vi "setUp.vi"(8 "error in (no error)":errorcluster, 11 "reference in":refnum<class "Instrument Addon Error System Tests.lvclass">) -> (0 "error out":errorcluster, 3 "reference out":refnum<class "Instrument Addon Error System Tests.lvclass">)   [LabVIEW 2020, in "Instrument Addon Error System Tests.lvclass"]
doc: "setUp runs prior to the test method during test execution. Use this method to initialize any object data required by your tests."
uses:
  Instrument Addon Error System Tests.lvclass
  C:/Program Files (x86)/National Instruments/LabVIEW 2020/vi.lib/NI/VeriStand Custom Device Testing Tools/VeriStandTestCase/VeriStandTestCase.lvclass
  C:/Program Files (x86)/National Instruments/LabVIEW 2020/vi.lib/addons/_JKI Toolkits/VI Tester/TestCase.llb/TestCase.lvclass
  <vilib>/addons/_JKI Toolkits/VI Tester/TestCase.llb/TestCase.lvclass
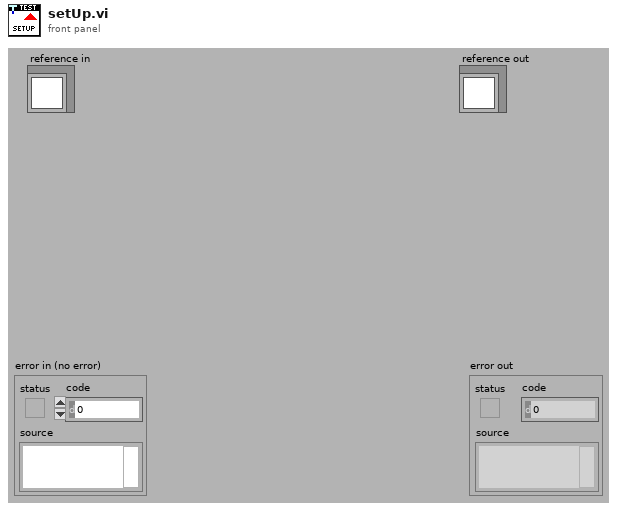
[diagram p1: front panel]
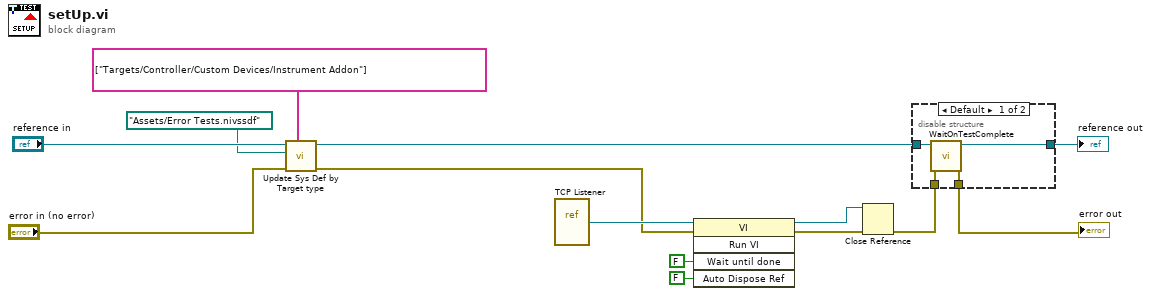
[diagram p0: block diagram]
diagram:
  n1 = call "Update Sys Def by Target type.vi"("nodepaths"=string[] ["Targets/Controller/Custom Devices/Instrument Addon"], "error in (no error)"="error in (no error)", "Sys Def relative path:"=path "Assets/Error Tests.nivssdf", "VeriStandTestCase in"="reference in") -> ("error out"=w3:errorcluster, "VeriStandTestCase out"=w5:refnum<class "Instrument Addon Error System Tests.lvclass">)  [unwired: 6 in]
  n2 = vi-ref "TCP Listener.vi"() -> (w12:refnum<vi>)
  n3 = invoke class="VI" method="Run VI"(reference=w12, error in=w3, "Wait until done"=FALSE ("Wait Until Done"), "Auto Dispose Ref"=FALSE ("Auto Dispose Reference")) -> (reference out=w11:refnum<vi>, error out=w10:errorcluster)  [unwired: 1 in, 3 out]
  n4 = Close Reference(reference=w11, error in (no error)=w10) -> (error out=w9:errorcluster)
  n5 = disable-structure shown="Default" {
    disable-tunnel: w9 -> [w18 w19]
    disable-tunnel: [w17 w19] -> w14
    disable-tunnel: [w16 w20] -> w13
    disable-tunnel: w5 -> [w15 w20]
    frame condition #0 (active) {
      n6 = call <vilib>:"WaitOnTestComplete.vi"("error in (no error)"=w18, "TestCase in"=w15) -> ("error out"=w17:errorcluster, "TestCase out"=w16:refnum<class "Instrument Addon Error System Tests.lvclass">)  [unwired: 8 in]
    }
    frame condition #1 {
    }
  }
  "error out" <- w14
  "reference out" <- w13
